vi "lvmcp_timeoutterm.vi"() -> ()   [LabVIEW 2015]
panel:
  out "error out":errorcluster
  out "terminal":refnum<vi>
  in  "reference":refnum<vi>
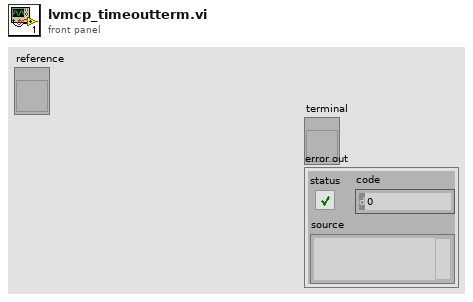
[diagram p1: front panel]
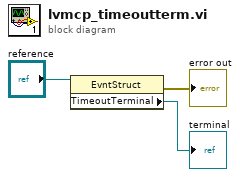
[diagram p0: block diagram]
diagram:
  n1 = property class="EvntStruct"(reference="reference") -> (error out=→"error out":errorcluster, "TimeoutTerminal"=→"terminal":refnum<vi>)  [unwired: 1 in, 1 out]
